vi "TrajectoryConfig_setCentripetalAccel.vi"(9 "Max Cent Accel":dbl format="%20.4f", 11 "inTRAJECTORY_CONFIG":T1 {"End Velocity" format="%20.4f"; "StartVelocity" format="%20.4f"; "Max Acceleration" format="%20.4f"; "MaxVelocity" format="%20.4f"}) -> (3 "outTRAJECTORY_CONFIG":T1 {"End Velocity" format="%20.4f"; "StartVelocity" format="%20.4f"; "Max Acceleration" format="%20.4f"; "MaxVelocity" format="%20.4f"})   [LabVIEW 2019, in "Trajectory_Library.lvlib"]
doc: "Adds and enables a centripital acceleration constraint to ensure that the rotating capability of the robot is not exceeded.\n\nParameters:\n - MaxCentAccel - The maximum centripetal acceleration (meters/sec^2)\n - InTrajectoryConfig - The trajectory configuration data structure\n\nReturns:\n - OutTrajectoryConfig - Modified trajectory configuration data structure\n modified to conain them."
uses:
  Trajectory_Library.lvlib
  TypeDef/TRAJ_CONFIG.ctl
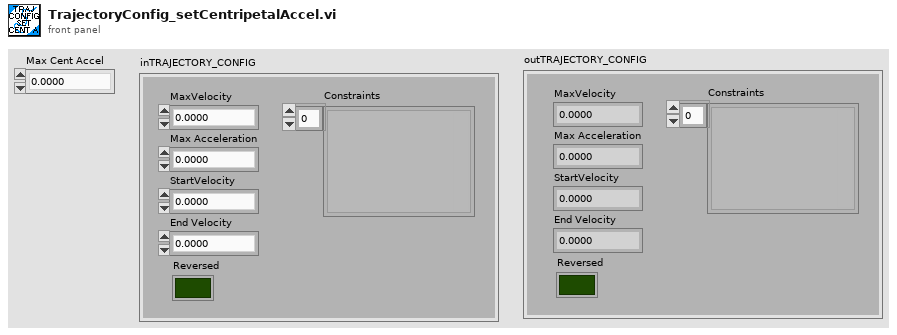
[diagram p1: front panel]
types:
  T1 = typedef "Trajectory_Library.lvlib/TRAJ_CONFIG.ctl" = cluster{"MaxVelocity":dbl, "Max Acceleration":dbl, "StartVelocity":dbl, "End Velocity":dbl, "Reversed":bool, "Constraints":variant[]}
  T2 = typedef "Trajectory_Library.lvlib/TRAJ_CONSTRAINT_CENTRIPETAL_ACCEL.ctl" = cluster{"Max Cent Accel":dbl}
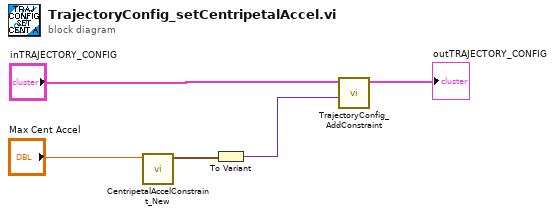
[diagram p0: block diagram]
diagram:
  n1 = call "CentripetalAccelConstraint_New.vi"("Max Cent Accel"="Max Cent Accel") -> ("CENTRIPETAL_ACCEL_CONSTRAINT"=w2:T2)  [unwired: 10 in]
  n2 = To Variant(anything=w2) -> (Variant=w4:variant)
  n3 = call "TrajectoryConfig_AddConstraint.vi"("Constraint"=w4, "inTRAJECTORY_CONFIG"="inTRAJECTORY_CONFIG") -> ("outTRAJECTORY_CONFIG"=→"outTRAJECTORY_CONFIG":T1)  [unwired: 9 in]
